vi "eDyno Load Torque.vi"(0 "Speed (rpm)":dbl, 5 "Speed Profile":T2={"Run-up Enabled"=FALSE, "Constant Speed (rpm)"=3000.0, "Run-up Start (rpm)"=500.0, "Run-up End (rpm)"=4500.0, "Run-up Duration (s)"=30.0}, 7 "Load Parameters":T1={"Base Torque T0 (Nm)"=0.2, "Drag Coeff k (Nm per rpm2)"=3e-08, "Rotor+Load Inertia J (kg m2)"=0.0005, "Max Torque (Nm)"=30.0}) -> (4 "Load Torque (Nm)":dbl)   [LabVIEW 2026]
doc: "PURPOSE\nSupplies the motor LOAD TORQUE that the eDyno NVH simulator does not produce, so the MCU_Status frame (0x300) carries a realistic torque instead of 0. Drop it in the CAN Status Generator Loop and wire Load Torque (Nm) into the Torque (Nm) element of the Status cluster of eDyno CAN Pack Signals.vi (which passes it to eDyno MCU Model.vi). Simple demo model - not a validated vehicle model.\n\nINPUTS\n- Speed (rpm): the simulator's Shaft Speed.\n- Speed Profile: the simulator's Speed Profile cluster (used to know whether a run-up is in progress and how fast it accelerates).\n- Load Parameters: drag and inertia coefficients. Defaults give about 0.2 Nm at standstill and about 0.8 Nm at 4500 rpm (typical e-bike mid-drive motor shaft before the gearbox).\n\nOUTPUT\n- Load Torque (Nm): positive = motoring. Limited to +/- Max Torque (and to the DBC range of MCU_TorqueEst, +/-32.767 Nm).\n\nEQUATIONS (one labelled frame each on the block diagram)\n1) T_drag = T0 + k x rpm^2 (rolling + aero-like drag seen by the motor)\n2) alpha = (Run-up End - Run-up Start)/Run-up Duration x 2pi/60 while a run-up is active and Speed < Run-up End, else 0; T_inertia = J x alpha\n3) Load Torque = T_drag + T_inertia, coerced to +/- Max Torque\n\nLIMITATIONS\nNo regen, no gear ratio, run-up acceleration assumed linear (matches the simulator's linear run-up). Duration is clamped to at least 0.1 s."
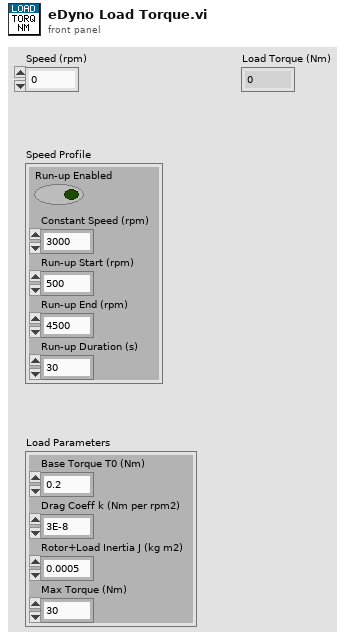
[diagram p1: front panel]
types:
  T1 = cluster{"Base Torque T0 (Nm)":dbl, "Drag Coeff k (Nm per rpm2)":dbl, "Rotor+Load Inertia J (kg m2)":dbl, "Max Torque (Nm)":dbl}
  T2 = cluster{"Run-up Enabled":bool, "Constant Speed (rpm)":dbl, "Run-up Start (rpm)":dbl, "Run-up End (rpm)":dbl, "Run-up Duration (s)":dbl}
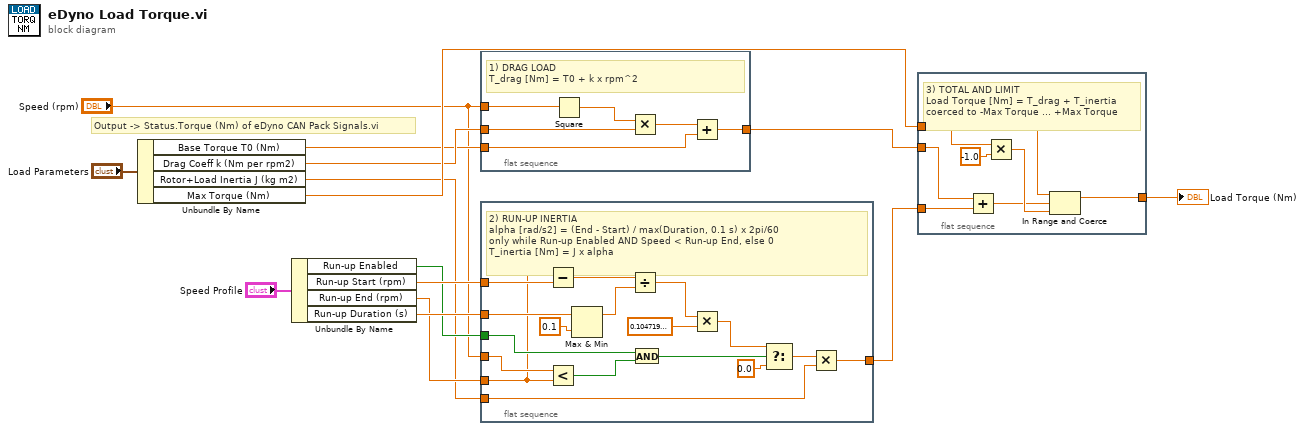
[diagram p0: block diagram]
diagram:
  # "Output -> Status.Torque (Nm) of eDyno CAN Pack Signals.vi"
  n1 = Unbundle By Name("Load Parameters") -> ("Base Torque T0 (Nm)"=w5:dbl, "Drag Coeff k (Nm per rpm2)"=w6:dbl, "Rotor+Load Inertia J (kg m2)"=w7:dbl, "Max Torque (Nm)"=w8:dbl)
  n2 = Unbundle By Name("Speed Profile") -> ("Run-up Enabled"=w9:bool, "Run-up Start (rpm)"=w10:dbl, "Run-up End (rpm)"=w11:dbl, "Run-up Duration (s)"=w12:dbl)
  n3 = flat-sequence {
    tunnel: "Speed (rpm)" -> [w16]
    tunnel: w5 -> [w20]
    tunnel: w6 -> [w18]
    tunnel: [w19] -> w13
    frame #0 {
      # "1) DRAG LOAD\nT_drag [Nm] = T0 + k x rpm^2"
      n4 = Square(x=w16) -> (x^2=w15:dbl)
      n5 = Multiply(x=w15, y=w18) -> (x*y=w17:dbl)
      n6 = Add(x=w17, y=w20) -> (x+y=w19:dbl)
    }
  }
  n7 = flat-sequence {
    tunnel: "Speed (rpm)" -> [w32]
    tunnel: w9 -> [w34]
    tunnel: w10 -> [w26]
    tunnel: w11 -> [w25]
    tunnel: w12 -> [w28]
    tunnel: w7 -> [w37]
    tunnel: [w36] -> w14
    frame #0 {
      # "2) RUN-UP INERTIA\nalpha [rad/s2] = (End - Start) / max(Duration, 0.1 s) x 2pi/60\nonly while Run-up Enabled AND Speed < Run-up End, else 0\nT_inertia [Nm] = J x alpha"
      n8 = Subtract(x=w25, y=w26) -> (x-y=w24:dbl)
      n9 = Less?(x=w32, y=w25) -> (x < y?=w31:bool)
      n10 = Max & Min(x=w28, y=0.1 ("min duration (s)")) -> (max(x,y)=w27:dbl)  [unwired: 1 out]
      n11 = Divide(x=w24, y=w27) -> (x/y=w29:dbl)
      n12 = And(x=w34, y=w31) -> (x .and. y?=w33:bool)
      n13 = Multiply(x=w29, y=0.10471975511965977 ("2pi/60 (rad/s per rpm)")) -> (x*y=w30:dbl)
      n14 = Select(t=w30, s=w33, f=0.0 ("no acceleration")) -> (s? t:f=w35:dbl)
      n15 = Multiply(x=w35, y=w37) -> (x*y=w36:dbl)
    }
  }
  n16 = flat-sequence {
    tunnel: w8 -> [w43]
    tunnel: w13 -> [w40]
    tunnel: w14 -> [w41]
    tunnel: [w44] -> w4
    frame #0 {
      # "3) TOTAL AND LIMIT\nLoad Torque [Nm] = T_drag + T_inertia\ncoerced to -Max Torque ... +Max Torque"
      n17 = Add(x=w40, y=w41) -> (x+y=w39:dbl)
      n18 = Multiply(x=w43, y=-1.0 ("minus one")) -> (x*y=w42:dbl)
      n19 = In Range and Coerce(upper limit=w43, x=w39, lower limit=w42) -> (coerced(x)=w44:dbl)  [unwired: 1 out]
    }
  }
  "Load Torque (Nm)" <- w4
